vi "Write to Data Source.vi"(7 "Project Store in":refnum<class "Project Store.lvclass">, 8 "error in (no error)":errorcluster) -> (0 "error out":errorcluster, 5 "Project Store out":refnum<class "Project Store.lvclass">)   [LabVIEW 2024, in "Project Store.lvclass"]
doc: "Saves the in-memory projects and tasks to the data source. The parent class has no data source and does nothing; children override it.\n\nGenerated by: Claude"
uses:
  Project Store.lvclass
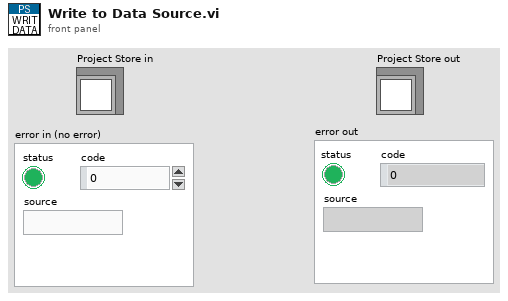
[diagram p1: front panel]
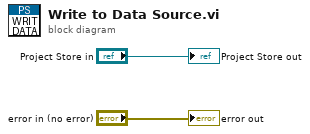
[diagram p0: block diagram]
diagram:
  "Project Store out" <- "Project Store in"
  "error out" <- "error in (no error)"
